vi "VIH Dialog - Project File Rules - Shortcut Menu Handler.vi"(6 "Menu Tag":string, 8 "Files":cluster{"Type":T1, "Path":path, "Lost":bool}[](array[cluster]), 10 "MenuRef":refnum<k9>, 11 "Event Type":T2) -> (3 "States spec":string)   [LabVIEW 2014]
doc: "::: VI Helpeks :::\nCopyright (c) 2000-2026 Konstantin Shifershteyn. All rights reserved."
uses:
  <vilib>/event_ctls.llb/lveventtype.ctl
  _VIH HelpGen - Palette.llb/VIH HelpGen Typedef - Palette - Item Type Enum.ctl
  _VIH Support Library.llb/VIH Utility - MENU - Create Menu (String).vi
panel:
  # "VI Helpeks\nCopyright (c) 2012-2026 Konstantin Shifershteyn"
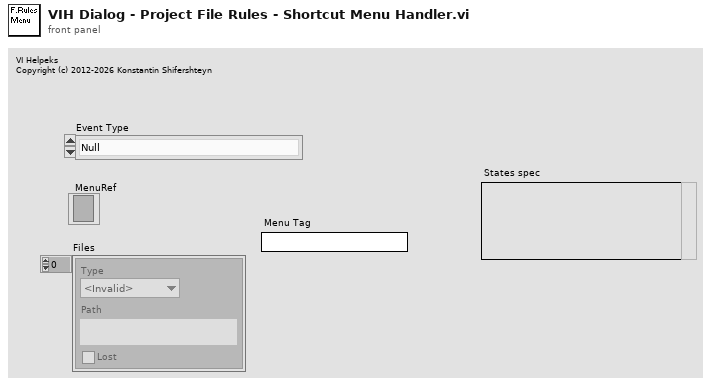
[diagram p1: front panel]
types:
  T1 = typedef "VIH HelpGen Typedef - Palette - Item Type Enum.ctl" = enum32{"<Invalid>", "<unknown>", "VI", "Menu", "LV Func", "Express VI", "Poly VI", "CTL", "HTML"}
  T2 = typedef "lveventtype.ctl" = enum32{"Null", "Timeout", "Annotation Menu Selection", "Annotation Menu Selection?", "App Instance Close", "App Instance Close?", "Autoscale Range Change", "Bookmark Info Change", "Cell Edit", "Cell Edit?", "Cursor Grab", "Cursor Grab?", "Cursor Menu Selection", "Cursor Menu Selection?", "Cursor Move", "Cursor Release", "Data Change", "Direction Change", "Display State Change", "Drag Ended", "Drag Enter", "Drag Leave", "Drag Over", "Drag Source Update", "Drag Starting", "Drag Starting?", "Drop", "Exec State Change", "Key Down", "Key Down?", "Key Repeat", "Key Repeat?", "Key Up", "Listbox Double Click", "Menu Activation?", "Menu Selection (App)", "Menu Selection? (App)", "Menu Selection (User)", "Mouse Down", "Mouse Down?", "Mouse Enter", "Mouse Leave", "Mouse Move", "Mouse Up", "Mouse Wheel", "NI Security User Change (App)", "Pane Size", "Panel Close", "Panel Close?", "Panel Resize", "Plot Attribute Change", "Scale Range Change", "Shortcut Menu Activation?", "Shortcut Menu Selection (App)", "Shortcut Menu Selection? (App)", "Shortcut Menu Selection (User)", "Tree Double Click", "Tree Drag", "Tree Drag?", "Tree Drop", "Tree Drop?", "Tree Item Close", "Tree Item Close?", "Tree Item Open", "Tree Item Open?", "User Event", "Value Change"}
  T3 = enum16{"get", "get all", "set", "Init", "delete", "rename"}
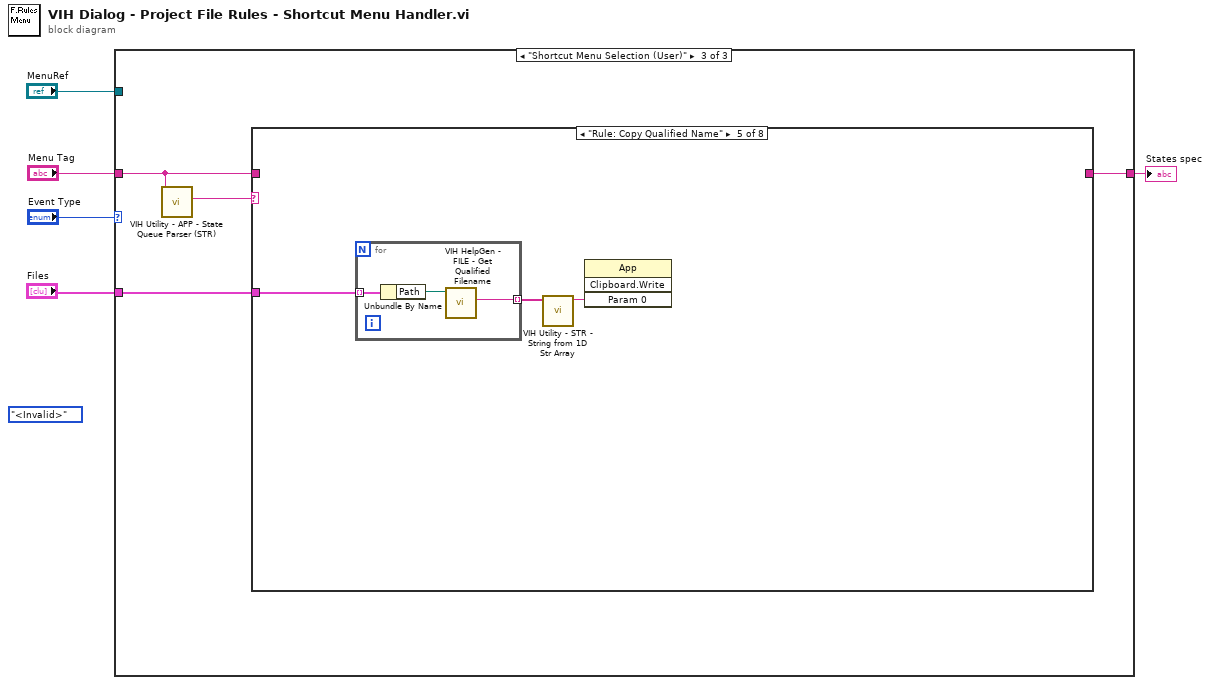
[diagram p0: block diagram]
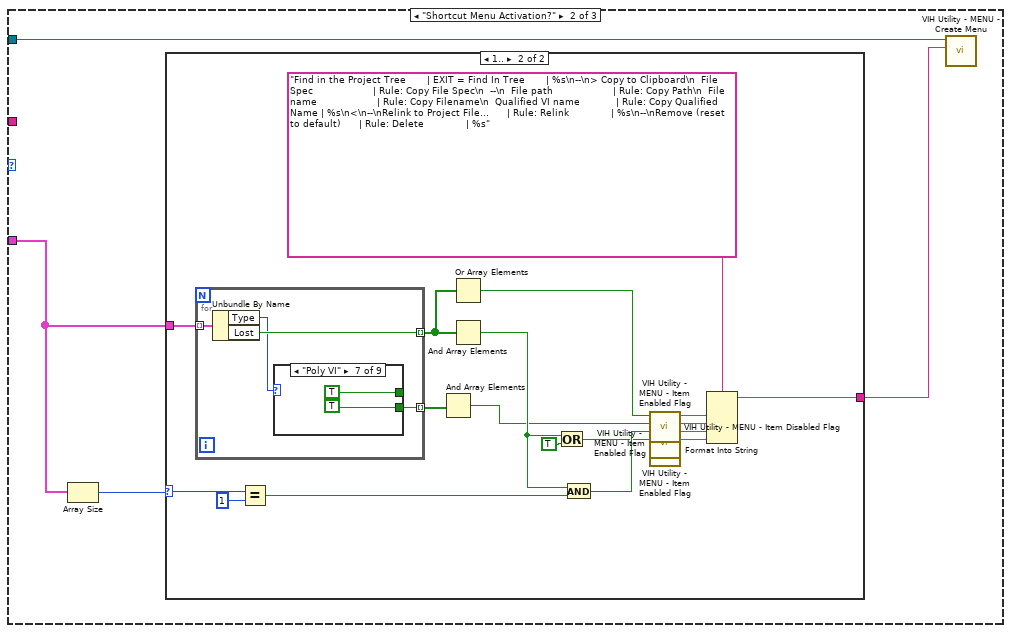
[diagram p3: hidden frame]
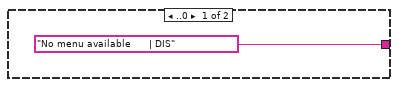
[diagram p4: hidden frame]
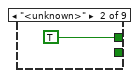
[diagram p6: hidden frame]
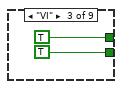
[diagram p7: hidden frame]
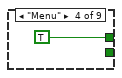
[diagram p8: hidden frame]
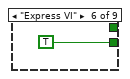
[diagram p10: hidden frame]
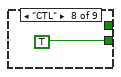
[diagram p11: hidden frame]
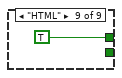
[diagram p12: hidden frame]
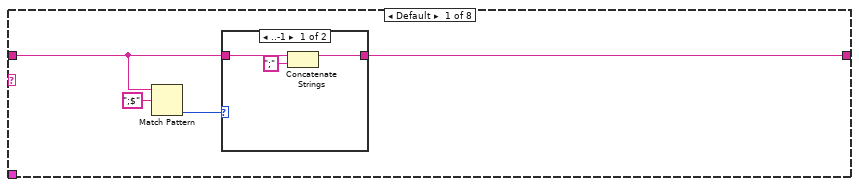
[diagram p13: hidden frame]
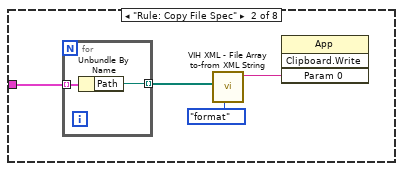
[diagram p15: hidden frame]
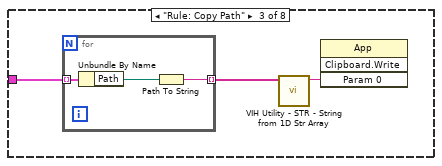
[diagram p16: hidden frame]
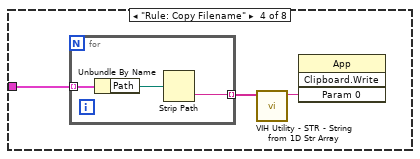
[diagram p17: hidden frame]
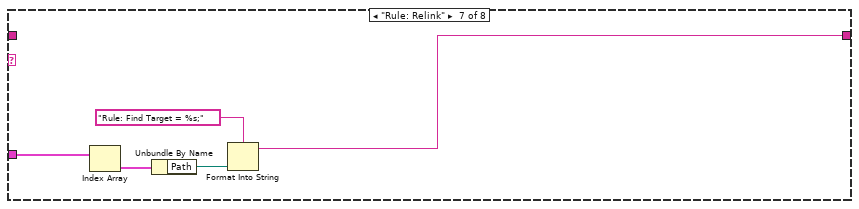
[diagram p19: hidden frame]
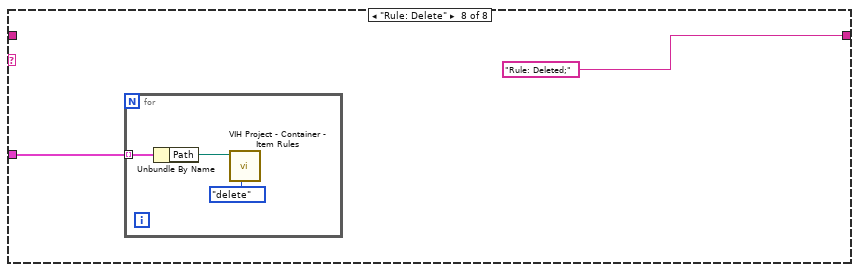
[diagram p20: hidden frame]
diagram:
  (unwired) VIH_HelpGen_Typedef_-_Palette_-_Item_Type_Enum."<Invalid>" ("Type")
  n1 = case shown="\"Shortcut Menu Selection (User)\"" "Event Type" {
    tunnel: "MenuRef" -> [_ w9 _]
    tunnel: [_ _ w43] -> w3
    tunnel: "Menu Tag" -> [_ _ w44]
    tunnel: "Files" -> [_ w6 w42]
    frame Default {
    }
    frame "Shortcut Menu Activation?" {
      n2 = Array Size(array=w6) -> (size(s)=w7:i32)
      n3 = case shown="1.." w7 {
        selector: w7 -> [_ w20]
        tunnel: ["No menu available      | DIS" w28] -> w8
        tunnel: w6 -> [_ w23]
        frame ..0 {
        }
        frame 1.. {
          n4 = for {
            tunnel: w23 -> [w32] mode=indexing
            tunnel: [w31] -> w21 mode=indexing
            tunnel: [w29] -> w13 mode=indexing
            n5 = Unbundle By Name(w32) -> ("Type"=w30:T1, "Lost"=w31:bool)
            n6 = case shown="\"Poly VI\"" w30 {
              tunnel: [_ TRUE TRUE TRUE _ _ TRUE _ TRUE] -> _
              tunnel: [_ _ TRUE _ _ TRUE TRUE TRUE _] -> w29
              frame "<Invalid>" {
              }
              frame "<unknown>" {
              }
              frame "VI" {
              }
              frame "Menu" {
              }
              frame "LV Func" {
              }
              frame "Express VI" {
              }
              frame "Poly VI" {
              }
              frame "CTL" {
              }
              frame "HTML" {
              }
            }
          }
          n7 = Equal?(x=w20, y=1) -> (x = y?=w18:bool)
          n8 = And Array Elements(Boolean array=w13) -> (logical AND=w12:bool)
          n9 = Or Array Elements(Boolean array=w21) -> (logical OR=w22:bool)
          n10 = And Array Elements(Boolean array=w21) -> (logical AND=w15:bool)
          n11 = Or(x=w15, y=TRUE) -> (x .or. y?=w16:bool)
          n12 = And(x=w15, y=w18) -> (x .and. y?=w17:bool)
          n13 = call "VIH Utility - MENU - Item Disabled Flag.vi"("Disable?"=w22) -> ("Disable flag"=w26:string)  [unwired: 10 in]
          n14 = call "VIH Utility - MENU - Item Enabled Flag.vi"("Enable?"=w12) -> ("Disable flag"=w11:string)  [unwired: 10 in]
          n15 = call "VIH Utility - MENU - Item Enabled Flag.vi"("Enable?"=w17) -> ("Disable flag"=w25:string)  [unwired: 10 in]
          n16 = call "VIH Utility - MENU - Item Enabled Flag.vi"("Enable?"=w16) -> ("Disable flag"=w24:string)  [unwired: 10 in]
          n17 = Format Into String(format string="Find in the Project Tree       | EXIT = Find In Tree       | %s\n--\n> Copy to Clipboard\n  File Spec                    | Rule: Copy File Spec\n  --\n  File path                    | Rule: Copy Path\n  File name                    | Rule: Copy Filename\n  Qualified VI name            | Rule: Copy Qualified Name | %s\n<\n--\nRelink to Project File...      | Rule: Relink              | %s\n--\nRemove (reset to default)      | Rule: Delete              | %s", w26, w11, w25, w24) -> (resulting string=w28:string)  [unwired: 2 in, 1 out]
        }
      }
      n18 = call-poly "VIH Utility - MENU - Create Menu.vi"("Menu Description"=w8, "menu"=w9) -> ()  [unwired: 8 in, 2 out]
    }
    frame "Shortcut Menu Selection (User)" {
      n19 = call "VIH Utility - APP - State Queue Parser (STR).vi"("input queue"=w44) -> ("state"=w45:string)  [unwired: 5 in, 3 out]
      n20 = case shown="\"Rule: Copy Qualified Name\"" w45 {
        tunnel: [w46 _ _ _ _ _ w78 "Rule: Deleted;" ("format string")] -> w43
        tunnel: w44 -> [w47 _ _ _ _ _ _ _]
        tunnel: w42 -> [_ w57 w61 w66 w72 _ w82 w83]
        frame Default {
          n21 = Match Pattern(string=w47, regular expression=";$") -> (offset past match=w48:i32)  [unwired: 1 in, 3 out]
          n22 = case shown="..-1" w48 {
            tunnel: w47 -> [w52 w53]
            tunnel: [w51 w53] -> w46
            frame ..-1 {
              n23 = Concatenate Strings(w52, ";" ("string")) -> (w51:string)
            }
            frame 0.. {
            }
          }
        }
        frame "Rule: Copy File Spec" {
          n24 = for {
            tunnel: w57 -> [w59] mode=indexing
            tunnel: [w58] -> w55 mode=indexing
            n25 = Unbundle By Name(w59) -> ("Path"=w58:path)
          }
          n26 = call "VIH XML - File Array to-from XML String.vi"("cmd (check)"=enum16{"check", "parse", "format"}."format", "Files in"=w55) -> ("XML out"=w54:string)  [unwired: 6 in, 3 out]
          n27 = invoke class="App" method="Clipboard.Write"("Param 0"=w54) -> ()  [unwired: 3 in, 4 out]
        }
        frame "Rule: Copy Path" {
          n28 = for {
            tunnel: w61 -> [w65] mode=indexing
            tunnel: [w64] -> w60 mode=indexing
            n29 = Unbundle By Name(w65) -> ("Path"=w63:path)
            n30 = Path To String(path=w63) -> (string=w64:string)
          }
          n31 = call "VIH Utility - STR - String from 1D Str Array.vi"("Array in"=w60) -> ("String out"=w62:string)  [unwired: 6 in]
          n32 = invoke class="App" method="Clipboard.Write"("Param 0"=w62) -> ()  [unwired: 3 in, 4 out]
        }
        frame "Rule: Copy Filename" {
          n33 = for {
            tunnel: [w71] -> w68 mode=indexing
            tunnel: w66 -> [w70] mode=indexing
            n34 = Unbundle By Name(w70) -> ("Path"=w69:path)
            n35 = Strip Path(path=w69) -> (name=w71:string)  [unwired: 1 out]
          }
          n36 = call "VIH Utility - STR - String from 1D Str Array.vi"("Array in"=w68) -> ("String out"=w67:string)  [unwired: 6 in]
          n37 = invoke class="App" method="Clipboard.Write"("Param 0"=w67) -> ()  [unwired: 3 in, 4 out]
        }
        frame "Rule: Copy Qualified Name" {
          n38 = for {
            tunnel: [w75] -> w73 mode=indexing
            tunnel: w72 -> [w77] mode=indexing
            n39 = Unbundle By Name(w77) -> ("Path"=w76:path)
            n40 = call "VIH HelpGen - FILE - Get Qualified Filename.vi"("File Path"=w76) -> ("Qualified name"=w75:string)  [unwired: 9 in, 1 out]
          }
          n41 = call "VIH Utility - STR - String from 1D Str Array.vi"("Array in"=w73) -> ("String out"=w74:string)  [unwired: 6 in]
          n42 = invoke class="App" method="Clipboard.Write"("Param 0"=w74) -> ()  [unwired: 3 in, 4 out]
        }
        frame "----------------------------- 1" {
        }
        frame "Rule: Relink" {
          n43 = Index Array(array=w82) -> (element=w81:cluster{"Type":T1, "Path":path, "Lost":bool})  [unwired: 1 in]
          n44 = Unbundle By Name(w81) -> ("Path"=w80:path)
          n45 = Format Into String(format string="Rule: Find Target = %s;", w80) -> (resulting string=w78:string)  [unwired: 2 in, 1 out]
        }
        frame "Rule: Delete" {
          n46 = for {
            tunnel: w83 -> [w87] mode=indexing
            n47 = Unbundle By Name(w87) -> ("Path"=w86:path)
            n48 = call "VIH Project - Container - Item Rules.vi"("cmd (get)"=T3."delete", "Item Path"=w86) -> ()  [unwired: 5 in, 5 out]
          }
        }
      }
    }
  }
  "States spec" <- w3
